vi "Sous_VI_trieur_couleur.vi"(6 "error in (no error)":errorcluster) -> (0 "error out":errorcluster, 3 "Couleur":bool)   [LabVIEW 2018]
uses:
  <vilib>/myRIO/Common/Instrument Driver Framework/Utilities/typedefs/Analog Scaling Constants.ctl
  <vilib>/myRIO/Common/Instrument Driver Framework/Utilities/typedefs/Analog Scaling Constants List.ctl
  <vilib>/myRIO/Common/Instrument Driver Framework/myRIO v1.0/AI/typedefs/AI Channels Enum.ctl
  <vilib>/myRIO/Common/Instrument Driver Framework/myRIO v1.0/AI/typedefs/AI Channels List.ctl
  <vilib>/myRIO/Common/Instrument Driver Framework/Utilities/typedefs/Generic FPGA Reference.ctl
  <vilib>/myRIO/Common/Instrument Driver Framework/Utilities/typedefs/myRIO v1.0 Reference.ctl
  <vilib>/myRIO/Common/Instrument Driver Framework/Utilities/typedefs/Hardware Version Enum.ctl
  <vilib>/myRIO/Common/Instrument Driver Framework/Utilities/typedefs/myRIO Generic Hardware Reference.ctl
  <vilib>/myRIO/Instrument Drivers/Onboard IO/AI/typedefs/AI Reference.ctl
  <vilib>/myRIO/Instrument Drivers/Onboard IO/AI/AI.lvlib
  <vilib>/myRIO/Instrument Drivers/Onboard IO/AI/vis/Read.vi
  <vilib>/myRIO/Instrument Drivers/Onboard IO/AI/vis/myRIO AI Open.xnode
  <vilib>/myRIO/Common/Instrument Driver Framework/Utilities/vis/Is FPGA Ref Available.vi
  <vilib>/myRIO/Express VI/Onboard IO/AI/AI Express VI.xnode
  <vilib>/myRIO/Common/Instrument Driver Framework/myRIO v1.0/AI/vis/myRIO v1.1 Open AI.vi
  <vilib>/userdefined/High Color/nirio_resource_hc.ctl
panel:
  out "Graphe déroulant":dbl(graph)
  out "Valeur capteur":sgl format="%#_3g"
  # "Détection du capteur couleur"
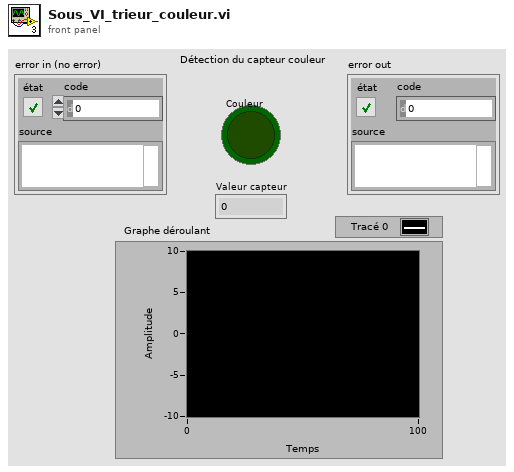
[diagram p1: front panel]
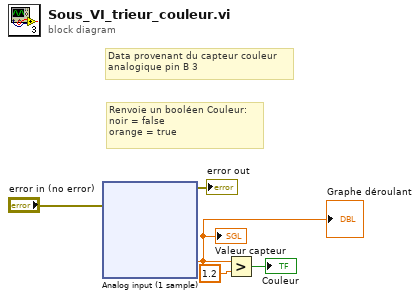
[diagram p0: block diagram]
diagram:
  # "Renvoie un booléen Couleur:\nnoir = false\norange = true"
  # "Data provenant du capteur couleur\nanalogique pin B 3"
  n1 = xnode "Analog input (1 sample)"("error in (no error)"="error in (no error)") -> ("Couleur (B/AI0 (Pin 3))"=w1:dbl, "error out"=→"error out":errorcluster)
  "Valeur capteur" <- w1
  "Graphe déroulant" <- w1
  n2 = Greater?(x=w1, y=1.2) -> (0:→"Couleur":bool)
